vi "Q_Greater_Order.vi"() -> ()   [LabVIEW 2026]
doc: "Use this template to build a VI to use as a subVI."
panel:
  out "x > y?":bool
  in  "Reading (bottom, y)":dbl
  in  "Threshold (top, x)":dbl
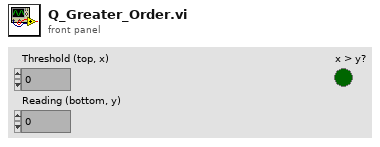
[diagram p1: front panel]
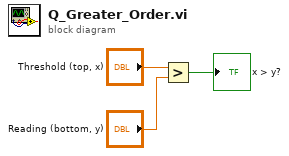
[diagram p0: block diagram]
diagram:
  n1 = Greater?(x="Threshold (top, x)", y="Reading (bottom, y)") -> (0:→"x > y?":bool)
